vi "Read Engine Reference.vi"(8 "error in (no error)":errorcluster, 11 "EasyUserManager in":refnum<class "EasyUserManager.lvclass">) -> (0 "error out":errorcluster, 2 "Engine Reference":refnum<k7>, 3 "EasyUserManager out":refnum<class "EasyUserManager.lvclass">)   [LabVIEW 2024, in "EasyUserManager.lvclass"]
doc: "Read the engine reference attribute of an EasyUserManager object.\n\nUse this VI (or the corresponding property node) to extract the engine reference for further usage in your code."
uses:
  EasyUserManager.lvclass
  EasyUserManager.lvclass/EasyUserManager.ctl
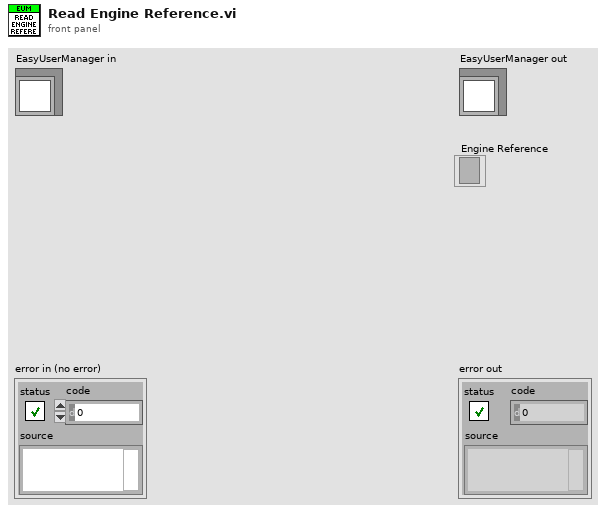
[diagram p1: front panel]
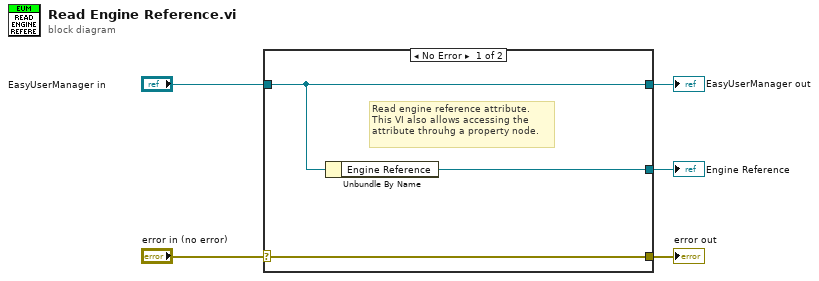
[diagram p0: block diagram]
diagram:
  n1 = case shown="No Error" "error in (no error)" {
    selector: "error in (no error)" -> [w8 w9]
    tunnel: [w8 w9] -> w4
    tunnel: [w7 w10] -> w2
    tunnel: "EasyUserManager in" -> [w7 w10]
    tunnel: [w6 _] -> w1
    frame No Error {
      # "Read engine reference attribute.\nThis VI also allows accessing the\nattribute throuhg a property node."
      n2 = Unbundle By Name(w7) -> ("Engine Reference"=w6:refnum<k7>)
    }
    frame Error {
      # "Pass error and do nothing."
    }
  }
  "error out" <- w4
  "EasyUserManager out" <- w2
  "Engine Reference" <- w1
